vi "Gserver_main.vi"(8 "Database location":path=path "D:/Sgraph_database", 10 "debug":bool, 11 "DAQ-Queue":refnum<queue>) -> ()   [LabVIEW 2020, in "Sgraph_lib_V1.lvlib" / "Gserver.lvclass"]
doc: "Gserver service.\n\nThis service will act on Gviewer queries.\nThis VI must be started to enable the Sgraph functionality\n\nUse the Close method of the Gserver class after the main application is ended to free all resources."
uses:
  Gserver.lvclass
  controls/Typedef_Gserver-init.ctl
  HISW/controls/typedef-DAQ-datagram.ctl
  HISW/controls/typedef-Qtype.ctl
  C:/Sgraph/Sgraph/source/Vsolver/Vsolver.lvclass
  Gserver.lvclass/Gserver.ctl
  Common/controls/MeMapInfo.ctl
  Common/controls/MMap_element.ctl
  FAMM/controls/typedef-functions.ctl
  Gview/controls/Typedef_Live.ctl
  controls/Typedef_Sgraph_Query.ctl
  Gview/controls/Typedef_Gserver-Replies.ctl
  Gview/controls/Typedef_ServerActions.ctl
  FAMM/FAMM.lvclass/FAMM.ctl
  Gview/controls/Typedef_datarequest.ctl
  FAMM/FAMM.lvclass
  HISW/HISW.lvclass
  FAMM/controls/typedef_FAMM_Query.ctl
  Common/controls/Global-services.vi
  Vsolver/Vsolver.lvclass
  Builds/Sgraph_lib_V1.lvlib
  Gview/Gviewer.lvclass
panel:
  out "error out":errorcluster
  out "HISW-# elements in queue":i32
  out "HISW-iteration":i32
  out "# elements in queue":i32
  out "Graphs Running":string[](array[string])
  out "Gserver":picture
  out "GserverInitState":T1
  # "debug info"
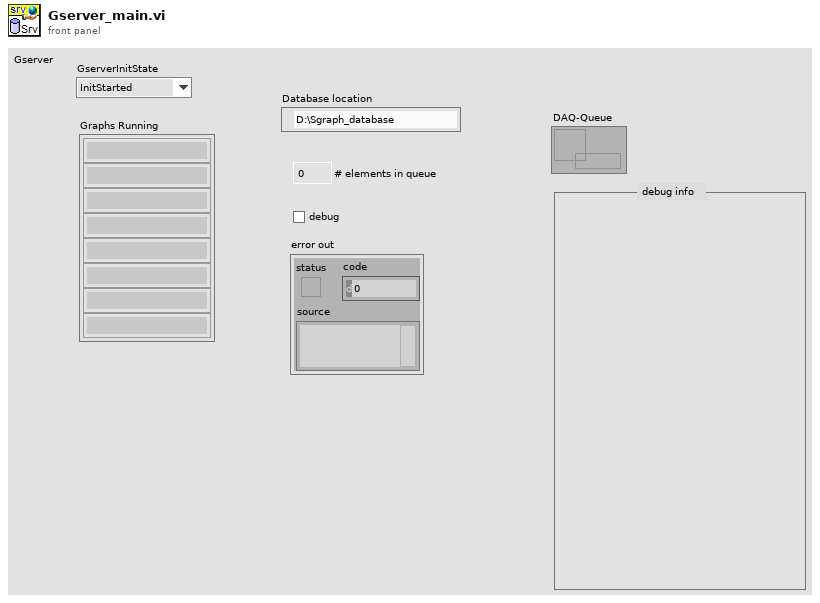
[diagram p1: front panel]
types:
  T1 = typedef "Sgraph_lib_V1.lvlib/Gserver.lvclass/Typedef_Gserver-init.ctl" = enum16{"InitStarted", "FAMM_started", "HISW_Started", "Active"}
  T2 = typedef "Sgraph_lib_V1.lvlib/typedef-functions.ctl" = enum16{"PAQ-request", "PAQ-taglist-request", "WAQ-request", "EAQ-request", "TAG-based-request", "PAQ-MemoryMap", "Exit-FAMM"}
  T3 = typedef "Sgraph_lib_V1.lvlib/MeMapInfo.ctl" = cluster{"MemLayer":T4[]}
  T4 = typedef "Sgraph_lib_V1.lvlib/MMap_element.ctl" = cluster{"Name":string, "Length":i32, "Pointer":i32, "Tbegin":dbl, "Tend":dbl, "Tmin":dbl, "Tmax":dbl, "Tpnt-1":dbl, "Tpnt":dbl, "Tpnt+1":dbl, "Array":dbl[]}
  T5 = typedef "Sgraph_lib_V1.lvlib/Gserver.lvclass/Typedef_Sgraph_Query.ctl" = cluster{"ViewportName":string, "Tags":string[], "Time-Start":timestamp, "Time-End":timestamp, "Pixels":i32, "Live":T6, "TimeSpan(sec)":dbl, "GViewer-Queue":refnum<queue>}
  T6 = typedef "Sgraph_lib_V1.lvlib/Gviewer.lvclass/Typedef_Live.ctl" = enum16{"Live View", "Freeze"}
  T7 = typedef "Sgraph_lib_V1.lvlib/Typedef_ServerActions.ctl" = enum16{"GraphUpdate", "SendAllTags", "SendIniPath", "SetGeneralOptions", "EditTagsOpen", "EditTagsPresetSave", "EditTagsPresetLoad", "EditTagsClose", "NewTagSelection", "ExitGraph"}
  T8 = typedef "Typedef_Gserver-Replies.ctl" = cluster{"ServerActions":T7, "data":variant, "Source":string, "Time Stamp":timestamp}
  T9 = typedef "Sgraph_lib_V1.lvlib/Gviewer.lvclass/Typedef_datarequest.ctl" = cluster{"Tags":string[], "Live":T6, "Time-Start":timestamp, "Time-End":timestamp, "TimeSpan":dbl, "DisplayResolution":i32}
  T10 = typedef "Sgraph_lib_V1.lvlib/typedef-Qtype.ctl" = enum16{"PAQ", "WAQ", "EAQ", "End-Service"}
  T11 = typedef "Sgraph_lib_V1.lvlib/typedef-DAQ-datagram.ctl" = cluster{"Time Stamp":timestamp, "Source":string, "Data":variant, "Qtype":T10}
  T12 = typedef "typedef_FAMM_Query.ctl" = cluster{"Time Stamp":timestamp, "FAMM-function":T2, "Source":string, "Data":variant}
  T13 = typedef "Sgraph_lib_V1.lvlib/Gserver.lvclass/Typedef_Gviewer-Query.ctl" = cluster{"Query_type":T14, "data":variant, "Source":string, "Time Stamp":timestamp}
  T14 = typedef "Sgraph_lib_V1.lvlib/Gserver.lvclass/Typedef_QueryType.ctl" = enum16{"Subscribe", "DataRequest", "RequestAllTags", "RequestIniPath", "FAMMstarted", "SetClientOptions", "GviewerUpdate", "OpenNewGraph", "CloseClient", "CloseAllClients", "Close Gserver", "OpenMemoryMap", "MeMapDataRequest", "MeMapDataResponse"}
  T15 = typedef "Sgraph_lib_V1.lvlib/FAMM.lvclass/Typedef_Gviewer_TagsUnits.ctl" = cluster{"PAQ_TAGs":string[], "WAQ_TAGs":string[], "EAQ_TAGs":string[], "PAQtagProps":T16[], "WAQtagProps":T16[], "EAQtagProps":T16[]}
  T16 = typedef "Sgraph_lib_V1.lvlib/typedef_com_TagProp.ctl" = cluster{"Description":string, "EngUnits":string, "RangeH":dbl, "RangeL":dbl, "Resolution":i32, "Obsolete":bool, "ChangeDate":timestamp, "ChangeSource":string, "ChangeReason":string, "TagFunc":u32}
  T17 = cluster{"FAMM_PAQ_Layers":i32, "FAMM_PAQ_resolution":dbl}
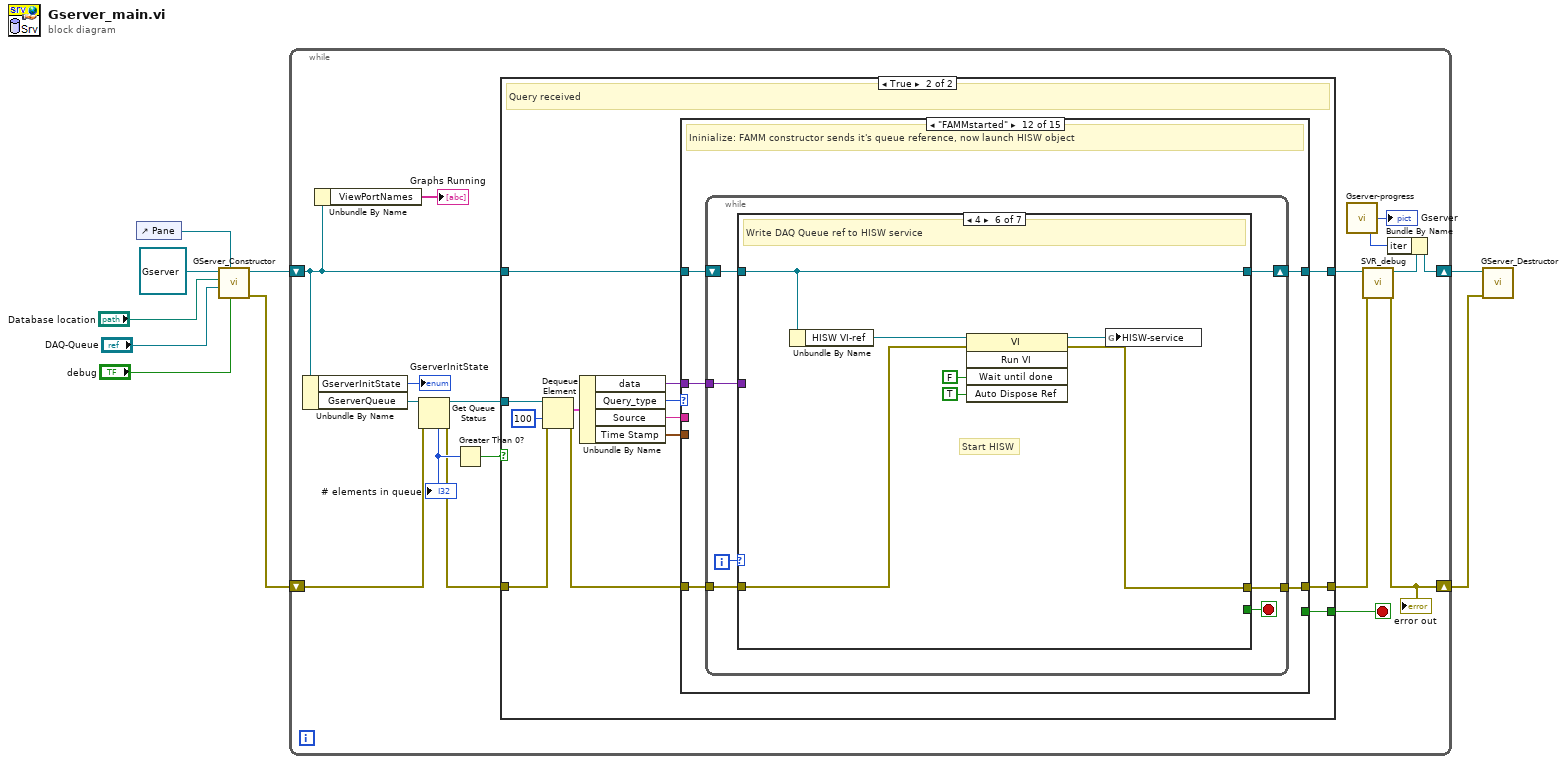
[diagram p0: block diagram]
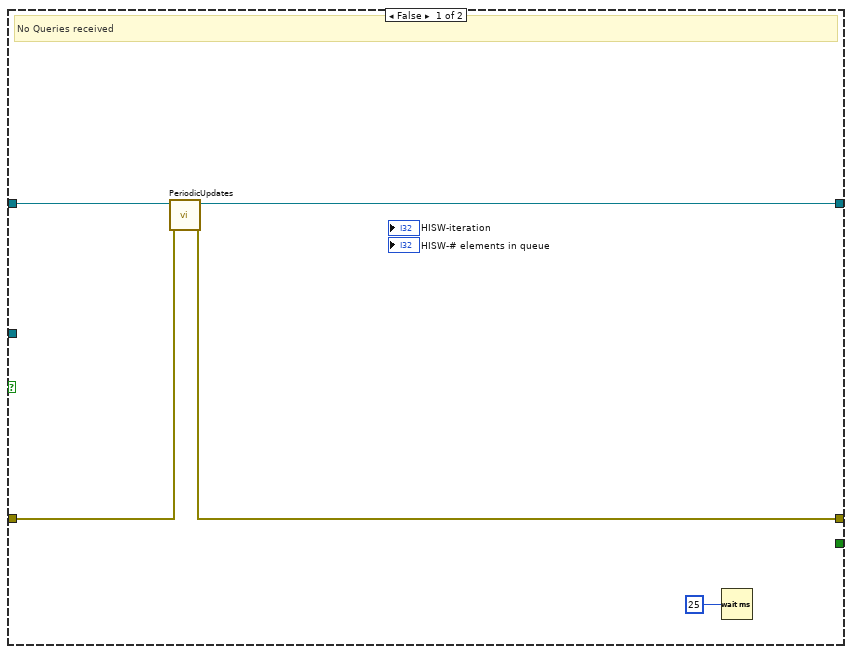
[diagram p2: hidden frame]
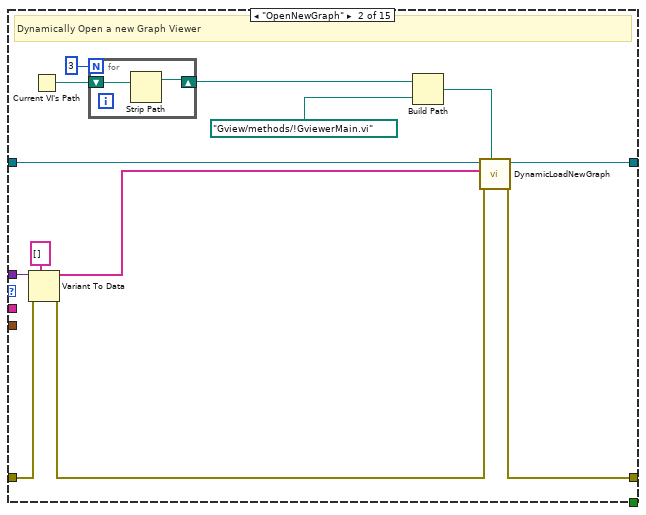
[diagram p4: hidden frame]
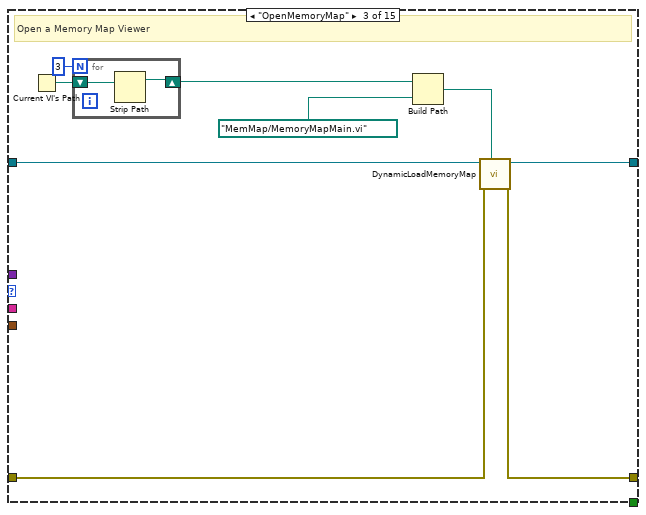
[diagram p5: hidden frame]
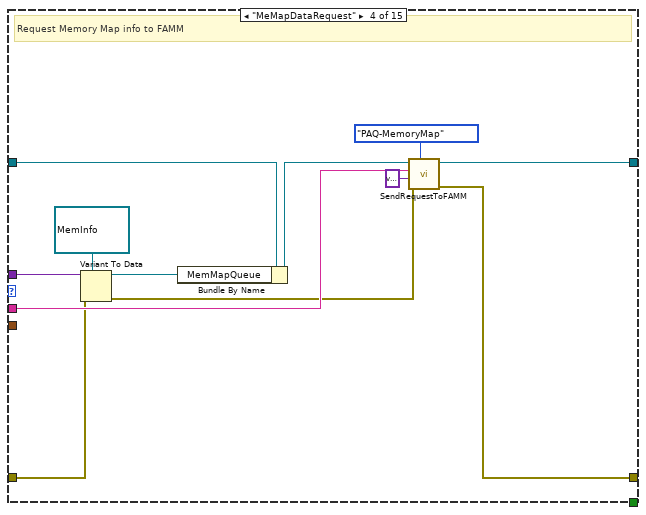
[diagram p6: hidden frame]
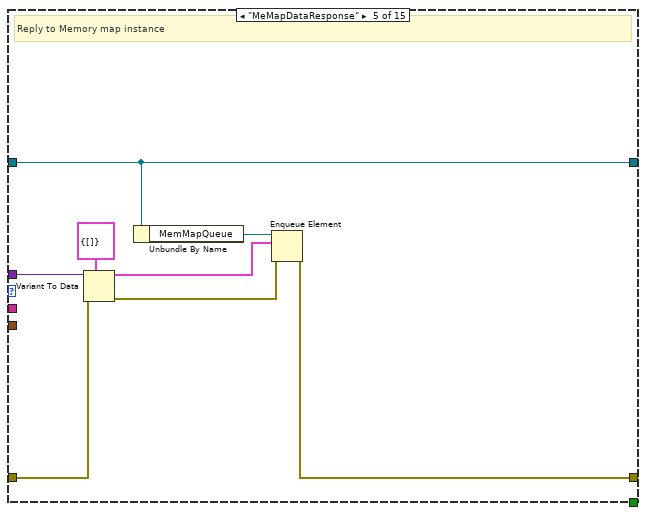
[diagram p7: hidden frame]
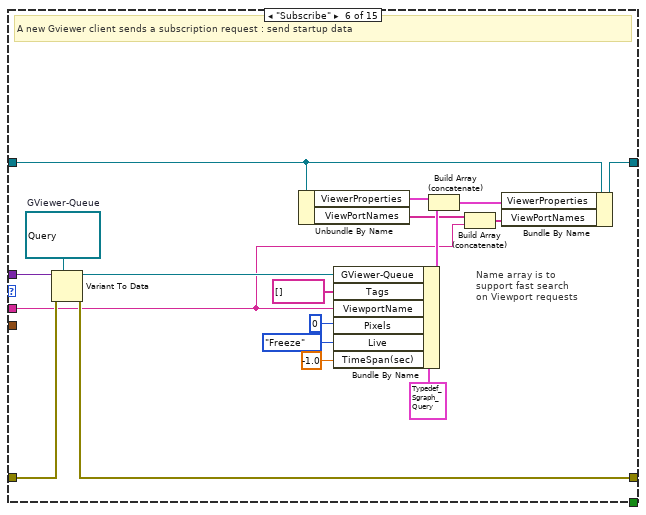
[diagram p8: hidden frame]
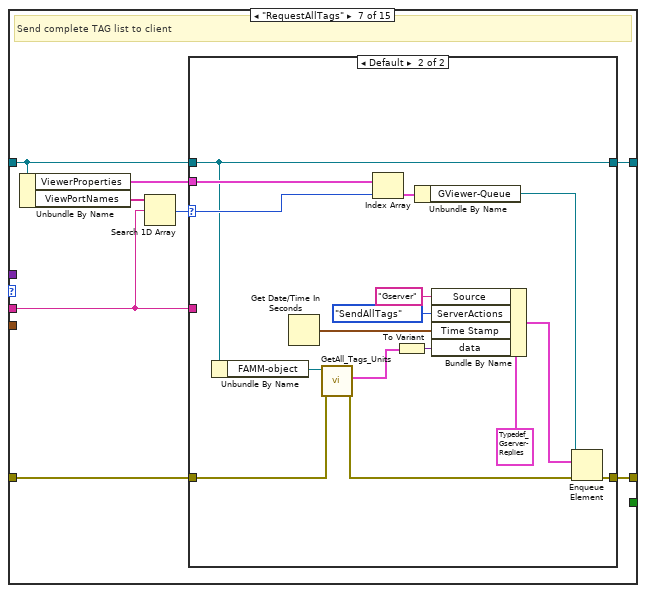
[diagram p9: hidden frame]
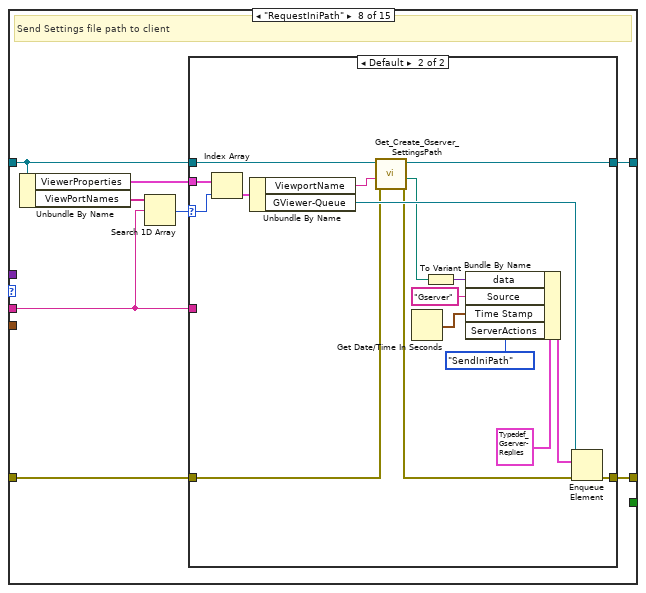
[diagram p11: hidden frame]
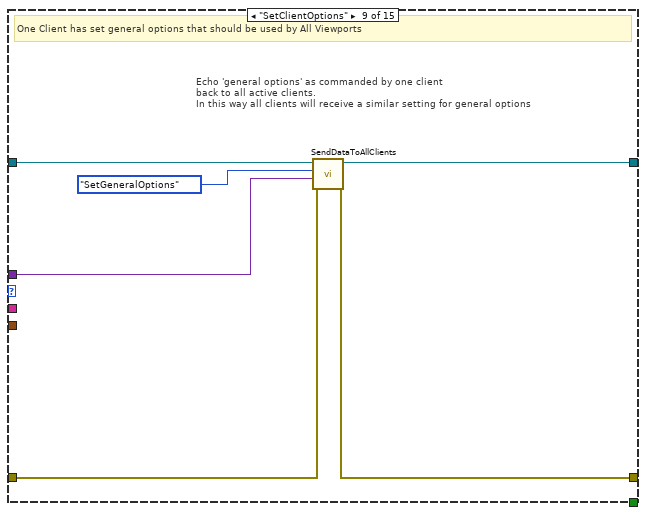
[diagram p13: hidden frame]
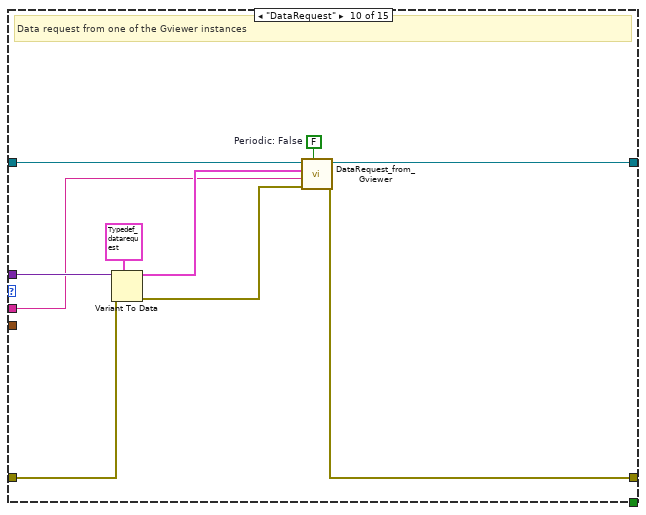
[diagram p14: hidden frame]
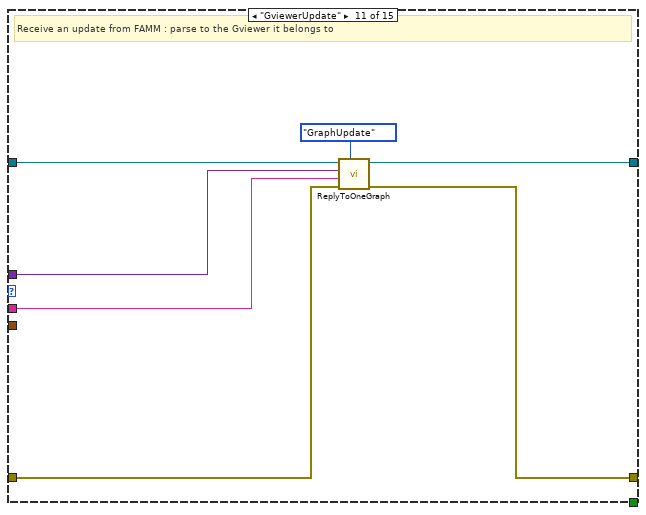
[diagram p15: hidden frame]
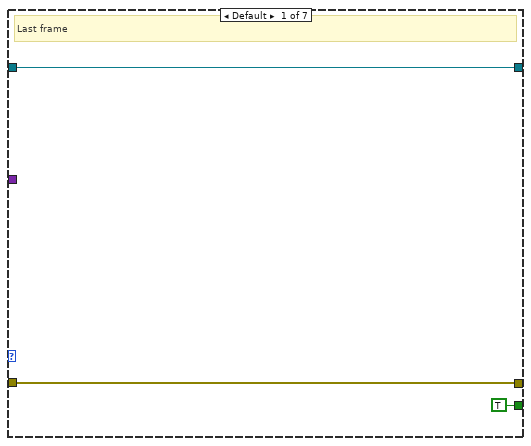
[diagram p16: hidden frame]
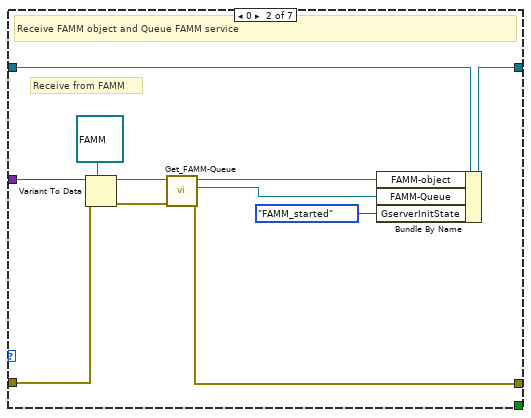
[diagram p17: hidden frame]
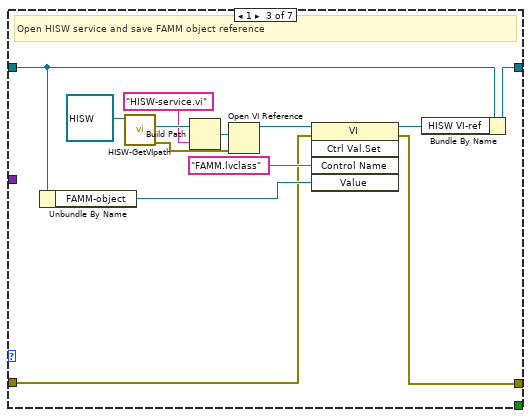
[diagram p18: hidden frame]
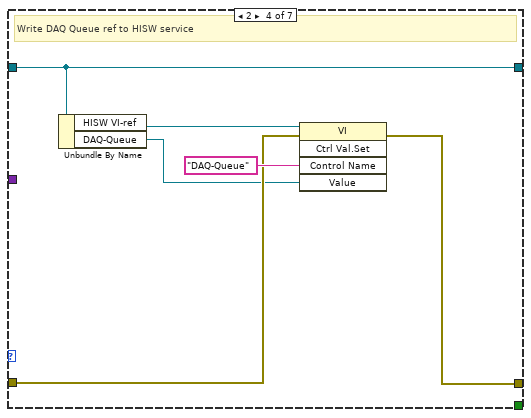
[diagram p19: hidden frame]
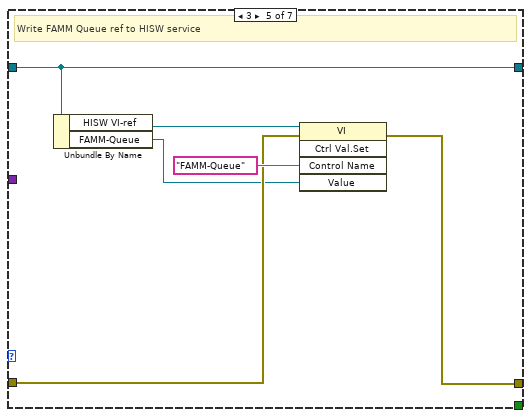
[diagram p20: hidden frame]
diagram:
  n1 = control-ref of="Pane"() -> (w1:refnum<vi>)
  n2 = call "GServer_Constructor.vi"("Debug"="debug", "Pane"=w1, "DAQ-Queue"="DAQ-Queue", "Database location"="Database location", "Gserver in"=refnum<class "Gserver.lvclass"> refnum) -> ("error out"=w8:errorcluster, "Gserver out"=w9:refnum<class "Gserver.lvclass">)  [unwired: 5 in]
  n3 = while {
    shift-right: [w15] -> w7
    shift-left: w9 -> [w17]
    shift-right: [w10] -> w6
    shift-left: w8 -> [w22]
    stop <- w18 stop-if-true
    n4 = Unbundle By Name(w17) -> ("GserverInitState"=→"GserverInitState":T1, "GserverQueue"=w26:refnum<queue>)
    n5 = Unbundle By Name(w17) -> ("ViewPortNames"=→"Graphs Running":string[])
    n6 = Get Queue Status(queue=w26, error in (no error)=w22) -> (queue out=w23:refnum<queue>, error out=w21:errorcluster, # elements in queue=w25:i32)  [unwired: 1 in, 5 out]
    "# elements in queue" <- w25
    n7 = Greater Than 0?(x=w25) -> (x > 0?=w24:bool)
    n8 = case shown="True" w24 {
      tunnel: w17 -> [w30 w38]
      tunnel: w21 -> [w29 w42]
      tunnel: [w28 w36] -> w13
      tunnel: [w27 w37] -> w11
      tunnel: w23 -> [_ w44]
      tunnel: [_ w33] -> w18
      frame False {
        # "No Queries received"
        n9 = call "PeriodicUpdates.vi"("error in (no error)"=w29, "Gserver in"=w30) -> ("error out"=w27:errorcluster, "Gserver out"=w28:refnum<class "Gserver.lvclass">)  [unwired: 8 in]
        n10 = Wait (ms)(milliseconds to wait=u32 25) -> ()  [unwired: 1 out]
      }
      frame True {
        # "Query received"
        n11 = Dequeue Element(queue=w44, timeout in ms (-1)=100, error in (no error)=w42) -> (element=w41:T13, error out=w39:errorcluster)  [unwired: 2 out]
        n12 = Unbundle By Name(w41) -> ("data"=w35:variant, "Query_type"=w40:T14, "Source"=w32:string, "Time Stamp"=w34:timestamp)
        n13 = case shown="\"FAMMstarted\"" w40 {
          tunnel: w39 -> [w45 w47 w63 w74 w85 w96 w114 w140 w165 w177 w182 w188 w255 w261 w272]
          tunnel: w38 -> [w46 w52 w65 w81 w92 w110 w116 w142 w169 w175 w186 w190 w257 w260 w271]
          tunnel: [w45 w51 w64 w75 w86 w97 w113 w139 w164 w171 w184 w187 w254 w258 w269] -> w37
          tunnel: [w46 w53 w66 w78 w92 w109 w115 w141 w168 w176 w185 w191 w256 w259 w270] -> w36
          tunnel: w35 -> [_ w59 _ w84 w90 w100 _ _ w166 w179 w180 w189 _ _ _]
          tunnel: w34 -> [_ _ _ _ _ _ _ _ _ _ _ _ _ _ _]
          tunnel: [_ _ _ _ _ _ _ _ _ _ _ _ _ _ w268] -> w33
          tunnel: w32 -> [_ _ _ w77 _ w93 w117 w143 _ w172 w183 _ w253 _ _]
          frame Default {
            # "Not implemented"
          }
          frame "OpenNewGraph" {
            # "Dynamically Open a new Graph Viewer"
            n14 = Variant To Data(error in=w47, type=string[] [], Variant=w59) -> (data=w49:string[], error out=w48:errorcluster)
            n15 = Current VI's Path() -> (path=w57:path)
            n16 = for {
              N: 3 -> [_]
              shift-right: [w60] -> w55
              shift-left: w57 -> [w61]
              n17 = Strip Path(path=w61) -> (stripped path=w60:path)  [unwired: 1 out]
            }
            n18 = Build Path(base path=w55, name or relative path=path "Gview/methods/!GviewerMain.vi") -> (appended path=w50:path)
            n19 = call "DynamicLoadNewGraph.vi"("ViewerPath"=w50, "error in (no error)"=w48, "Preferred_tags"=w49, "Gserver in"=w52) -> ("error out"=w51:errorcluster, "Gserver out"=w53:refnum<class "Gserver.lvclass">)  [unwired: 6 in]
          }
          frame "OpenMemoryMap" {
            # "Open a Memory Map Viewer"
            n20 = Current VI's Path() -> (path=w70:path)
            n21 = for {
              N: 3 -> [_]
              shift-right: [w71] -> w68
              shift-left: w70 -> [w72]
              n22 = Strip Path(path=w72) -> (stripped path=w71:path)  [unwired: 1 out]
            }
            n23 = Build Path(base path=w68, name or relative path=path "MemMap/MemoryMapMain.vi") -> (appended path=w62:path)
            n24 = call "DynamicLoadMemoryMap.vi"("ApplicationPath"=w62, "error in (no error)"=w63, "Gserver in"=w65) -> ("error out"=w64:errorcluster, "Gserver out"=w66:refnum<class "Gserver.lvclass">)  [unwired: 7 in]
          }
          frame "MeMapDataRequest" {
            # "Request Memory Map info to FAMM"
            n25 = Variant To Data(error in=w74, type=refnum<queue> refnum ("queue out"), Variant=w84) -> (data=w82:refnum<queue>, error out=w76:errorcluster)
            n26 = Bundle By Name(cluster=w81, "MemMapQueue"=w82) -> (w79:refnum<class "Gserver.lvclass">)
            n27 = call "SendRequestToFAMM.vi"("FAMM-function"=typedef-functions."PAQ-MemoryMap", "error in (no error)"=w76, "Data"=variant, "Source"=w77, "Gserver in"=w79) -> ("error out"=w75:errorcluster, "Gserver out"=w78:refnum<class "Gserver.lvclass">)  [unwired: 5 in]
          }
          frame "MeMapDataResponse" {
            # "Reply to Memory map instance"
            n28 = Variant To Data(error in=w85, type=T3 {"MemLayer"=[]} ("element"), Variant=w90) -> (data=w87:T3, error out=w88:errorcluster)
            n29 = Unbundle By Name(w92) -> ("MemMapQueue"=w91:refnum<queue>)
            n30 = Enqueue Element(queue=w91, element=w87, error in (no error)=w88) -> (error out=w86:errorcluster)  [unwired: 1 in, 2 out]
          }
          frame "Subscribe" {
            w101 = refnum<queue> refnum  # GViewer-Queue
            # "Name array is to\nsupport fast search\non Viewport requests"
            # "A new Gviewer client sends a subscription request : send startup data"
            n31 = Variant To Data(error in=w96, type=w101, Variant=w100) -> (data=w99:refnum<queue>, error out=w97:errorcluster)
            n32 = Unbundle By Name(w110) -> ("ViewerProperties"=w108:T5[], "ViewPortNames"=w95:string[])
            n33 = Bundle By Name(cluster=T5 {"ViewportName"="", "Tags"=[], "Time-Start"=timestamp(0 s since 1904-01-01), "Time-End"=timestamp(0 s since 1904-01-01), "Pixels"=0, "Live"=enum."Live View", "TimeSpan(sec)"=0.0, "GViewer-Queue"=refnum} ("Query_datagram"), "GViewer-Queue"=w99, "Tags"=string[] [], "ViewportName"=w93, "Pixels"=0, "Live"=Typedef_Live."Freeze", "TimeSpan(sec)"=-1.0) -> (w105:T5)
            n34 = Build Array (concatenate)(w108, w105) -> (w107:T5[])
            n35 = Build Array (concatenate)(w95, w93) -> (w94:string[])
            n36 = Bundle By Name(cluster=w110, "ViewerProperties"=w107, "ViewPortNames"=w94) -> (w109:refnum<class "Gserver.lvclass">)
          }
          frame "RequestAllTags" {
            # "Send complete TAG list to client"
            n37 = Unbundle By Name(w116) -> ("ViewerProperties"=w112:T5[], "ViewPortNames"=w118:string[])
            n38 = Search 1D Array(1D array=w118, element=w117) -> (index of element=w111:i32)  [unwired: 1 in]
            n39 = case shown="Default" w111 {
              selector: w111 -> [_ w135]
              tunnel: w117 -> [_ _]
              tunnel: w116 -> [w120 w131]
              tunnel: [w120 w131] -> w115
              tunnel: w114 -> [w119 w123]
              tunnel: [w119 w132] -> w113
              tunnel: w112 -> [_ w136]
              frame -1 {
              }
              frame Default {
                n40 = Unbundle By Name(w131) -> ("FAMM-object"=w124:refnum<class "FAMM.lvclass">)
                n41 = Get Date/Time In Seconds() -> (seconds since 1Jan1904=w127:timestamp)
                n42 = call "GetAll_Tags_Units.vi"("error in (no error)"=w123, "FAMM in"=w124) -> ("error out"=w122:errorcluster, "Tags_Units"=w121:T15)  [unwired: 7 in, 1 out]
                n43 = Index Array(array=w136, index=w135) -> (element=w134:T5)
                n44 = To Variant(anything=w121) -> (Variant=w125:variant)
                n45 = Unbundle By Name(w134) -> ("GViewer-Queue"=w133:refnum<queue>)
                n46 = Bundle By Name(cluster=T8 {"ServerActions"=enum."GraphUpdate", "data"=variant, "Source"="", "Time Stamp"=timestamp(0 s since 1904-01-01)} ("element"), "Source"="Gserver", "ServerActions"=Typedef_ServerActions."SendAllTags", "Time Stamp"=w127, "data"=w125) -> (w129:T8)
                n47 = Enqueue Element(queue=w133, element=w129, error in (no error)=w122) -> (error out=w132:errorcluster)  [unwired: 1 in, 2 out]
              }
            }
          }
          frame "RequestIniPath" {
            # "Send Settings file path to client"
            n48 = Unbundle By Name(w142) -> ("ViewerProperties"=w138:T5[], "ViewPortNames"=w144:string[])
            n49 = Search 1D Array(1D array=w144, element=w143) -> (index of element=w137:i32)  [unwired: 1 in]
            n50 = case shown="Default" w137 {
              selector: w137 -> [_ w162]
              tunnel: w143 -> [_ _]
              tunnel: w142 -> [w146 w154]
              tunnel: [w146 w155] -> w141
              tunnel: w140 -> [w145 w151]
              tunnel: [w145 w159] -> w139
              tunnel: w138 -> [_ w163]
              frame -1 {
              }
              frame Default {
                n51 = Index Array(array=w163, index=w162) -> (element=w161:T5)
                n52 = Unbundle By Name(w161) -> ("ViewportName"=w153:string, "GViewer-Queue"=w160:refnum<queue>)
                n53 = call "Get_Create_Gserver_SettingsPath.vi"("error in (no error)"=w151, "ViewPortName"=w153, "Gserver in"=w154) -> ("error out"=w152:errorcluster, "Viewport settings path"=w147:path, "Gserver out"=w155:refnum<class "Gserver.lvclass">)  [unwired: 6 in]
                n54 = Get Date/Time In Seconds() -> (seconds since 1Jan1904=w149:timestamp)
                n55 = To Variant(anything=w147) -> (Variant=w150:variant)
                n56 = Bundle By Name(cluster=T8 {"ServerActions"=enum."GraphUpdate", "data"=variant, "Source"="", "Time Stamp"=timestamp(0 s since 1904-01-01)} ("element"), "data"=w150, "Source"="Gserver", "Time Stamp"=w149, "ServerActions"=Typedef_ServerActions."SendIniPath") -> (w157:T8)
                n57 = Enqueue Element(queue=w160, element=w157, error in (no error)=w152) -> (error out=w159:errorcluster)  [unwired: 1 in, 2 out]
              }
            }
          }
          frame "SetClientOptions" {
            # "Echo 'general options' as commanded by one client\nback to all active clients.\nIn this way all clients will receive a similar setting for general options"
            # "One Client has set general options that should be used by All Viewports"
            n58 = call "SendDataToAllClients.vi"("error in (no error)"=w165, "data"=w166, "ServerActions"=Typedef_ServerActions."SetGeneralOptions", "Gserver in"=w169) -> ("error out"=w164:errorcluster, "Gserver out"=w168:refnum<class "Gserver.lvclass">)  [unwired: 6 in]
          }
          frame "DataRequest" {
            w170 = FALSE  # Periodic: False
            # "Data request from one of the Gviewer instances"
            n59 = Variant To Data(error in=w177, type=T9 {"Tags"=[], "Live"=enum."Live View", "Time-Start"=timestamp(0 s since 1904-01-01), "Time-End"=timestamp(0 s since 1904-01-01), "TimeSpan"=0.0, "DisplayResolution"=0} ("Cluster"), Variant=w179) -> (data=w174:T9, error out=w173:errorcluster)
            n60 = call "DataRequest_from_Gviewer.vi"("Periodic?"=w170, "error in (no error)"=w173, "Sending Gviewer"=w172, "DataRequest"=w174, "Gserver in"=w175) -> ("error out"=w171:errorcluster, "Gserver out"=w176:refnum<class "Gserver.lvclass">)  [unwired: 5 in]
          }
          frame "GviewerUpdate" {
            # "Receive an update from FAMM : parse to the Gviewer it belongs to"
            n61 = call "ReplyToOneGraph.vi"("ServerActions"=Typedef_ServerActions."GraphUpdate", "error in (no error)"=w182, "Graph name"=w183, "data"=w180, "Gserver in"=w186) -> ("error out"=w184:errorcluster, "Gserver out"=w185:refnum<class "Gserver.lvclass">)  [unwired: 5 in]
          }
          frame "FAMMstarted" {
            # "Ininialize: FAMM constructor sends it's queue reference, now launch HISW object"
            n62 = while {
              tunnel: w189 -> [w196]
              tunnel: w188 -> [w195]
              shift-right: [w198] -> w191
              shift-left: w190 -> [w197]
              tunnel: [w192] -> w187
              i -> [w194]
              stop <- w193 stop-if-true
              n63 = case shown="4" w194 {
                tunnel: [w201 w212 w215 w229 w235 w244 w246] -> w198
                tunnel: w197 -> [w201 w210 w214 w229 w235 w244 w245]
                tunnel: w196 -> [_ w209 _ _ _ _ _]
                tunnel: w195 -> [w199 w208 w217 w230 w236 w240 w250]
                tunnel: [TRUE _ _ _ _ _ _] -> w193
                tunnel: [w199 w204 w213 w226 w232 w239 w251] -> w192
                frame Default {
                  # "Last frame"
                }
                frame 0 {
                  # "Receive from FAMM"
                  # "Receive FAMM object and Queue FAMM service"
                  n64 = Variant To Data(error in=w208, type=refnum<class "FAMM.lvclass"> refnum ("FAMM out"), Variant=w209) -> (data=w206:refnum<class "FAMM.lvclass">, error out=w205:errorcluster)
                  n65 = call-dynamic "Get_FAMM-Queue.vi"("error in (no error)"=w205, "FAMM in"=w206) -> ("error out"=w204:errorcluster, "FAMM-Queue"=w202:refnum<queue>, "FAMM out"=w203:refnum<class "FAMM.lvclass">)  [unwired: 7 in]
                  n66 = Bundle By Name(cluster=w210, "FAMM-object"=w203, "FAMM-Queue"=w202, "GserverInitState"=Typedef_Gserver-init."FAMM_started") -> (w212:refnum<class "Gserver.lvclass">)
                }
                frame 1 {
                  # "Open HISW service and save FAMM object reference"
                  n67 = Unbundle By Name(w214) -> ("FAMM-object"=w218:refnum<class "FAMM.lvclass">)
                  n68 = call "HISW-GetVIpath.vi"("HISW in"=refnum<class "HISW.lvclass"> refnum) -> ("error out"=w223:errorcluster, "MethodsPath"=w224:path)  [unwired: 8 in, 1 out]
                  n69 = Build Path(base path=w224, name or relative path="HISW-service.vi") -> (appended path=w225:path)
                  n70 = Open VI Reference(vi path=w225, error in (no error)=w223) -> (vi reference=w222:refnum<vi>)  [unwired: 4 in, 1 out]
                  n71 = invoke class="VI" method="Ctrl Val.Set"(reference=w222, error in=w217, "Control Name"="FAMM.lvclass", "Value"=w218) -> (reference out=w216:refnum<vi>, error out=w213:errorcluster)  [unwired: 1 in, 3 out]
                  n72 = Bundle By Name(cluster=w214, "HISW VI-ref"=w216) -> (w215:refnum<class "Gserver.lvclass">)
                }
                frame 2 {
                  # "Write DAQ Queue ref to HISW service"
                  n73 = Unbundle By Name(w229) -> ("HISW VI-ref"=w228:refnum<vi>, "DAQ-Queue"=w227:refnum<queue>)
                  n74 = invoke class="VI" method="Ctrl Val.Set"(reference=w228, error in=w230, "Control Name"="DAQ-Queue", "Value"=w227) -> (error out=w226:errorcluster)  [unwired: 1 in, 4 out]
                }
                frame 3 {
                  # "Write FAMM Queue ref to HISW service"
                  n75 = Unbundle By Name(w235) -> ("HISW VI-ref"=w234:refnum<vi>, "FAMM-Queue"=w233:refnum<queue>)
                  n76 = invoke class="VI" method="Ctrl Val.Set"(reference=w234, error in=w236, "Control Name"="FAMM-Queue", "Value"=w233) -> (error out=w232:errorcluster)  [unwired: 1 in, 4 out]
                }
                frame 4 {
                  # "Start HISW"
                  # "Write DAQ Queue ref to HISW service"
                  n77 = Unbundle By Name(w244) -> ("HISW VI-ref"=w241:refnum<vi>)
                  n78 = invoke class="VI" method="Run VI"(reference=w241, error in=w240, "Wait until done"=FALSE ("Wait Until Done"), "Auto Dispose Ref"=TRUE ("Auto Dispose Reference")) -> (reference out=w238:refnum<vi>, error out=w239:errorcluster)  [unwired: 1 in, 3 out]
                  n79 = global write "Global-services.vi" "HISW-service"(w238) -> ()
                }
                frame 5 {
                  # "Get FAMM PAQ resolution data"
                  n80 = Unbundle By Name(w245) -> ("FAMM-object"=w252:refnum<class "FAMM.lvclass">)
                  n81 = call "GetPAQresolution.vi"("error in (no error)"=w250, "FAMM in"=w252) -> ("error out"=w251:errorcluster, "PAQ-resolution"=w249:T17)  [unwired: 7 in, 1 out]
                  n82 = Unbundle By Name(w249) -> ("FAMM_PAQ_Layers"=w248:i32, "FAMM_PAQ_resolution"=w247:dbl)
                  n83 = Bundle By Name(cluster=w245, "FAMM_PAQ_Layers"=w248, "FAMM_PAQ_resolution"=w247) -> (w246:refnum<class "Gserver.lvclass">)
                }
              }
            }
          }
          frame "CloseClient" {
            # "Graph display request to close the graph"
            n84 = call "CloseOneGraph.vi"("error in (no error)"=w255, "Graph name"=w253, "Gserver in"=w257) -> ("error out"=w254:errorcluster, "Gserver out"=w256:refnum<class "Gserver.lvclass">)  [unwired: 7 in]
          }
          frame "CloseAllClients" {
            # "One Graph display requests to close all Graphs"
            n85 = Unbundle By Name(w260) -> ("ViewPortNames"=w262:string[])
            n86 = for "Loop over all viewports and perform a clean Graph Close" {
              tunnel: w262 -> [w266] mode=indexing
              shift-right: [w263] -> w259
              shift-left: w260 -> [w267]
              shift-right: [w264] -> w258
              shift-left: w261 -> [w265]
              n87 = call "CloseOneGraph.vi"("error in (no error)"=w265, "Graph name"=w266, "Gserver in"=w267) -> ("error out"=w264:errorcluster, "Gserver out"=w263:refnum<class "Gserver.lvclass">)  [unwired: 7 in]
            }
          }
          frame "Close Gserver" {
            # "Close the SGraph server"
            n88 = while {
              shift-right: [w276] -> w269
              shift-left: w272 -> [w277]
              shift-right: [w274] -> w270
              shift-left: w271 -> [w275]
              tunnel: [w273] -> w268
              i -> [w278]
              stop <- w273 stop-if-true
              n89 = case shown="1" w278 {
                tunnel: [TRUE _ _ _] -> w273
                tunnel: w277 -> [w280 w291 w299 w302]
                tunnel: [w280 w289 w298 w303] -> w276
                tunnel: w275 -> [w279 w292 w301 w305]
                tunnel: [w279 w283 w301 w306] -> w274
                frame Default {
                  # "Last frame: no code here"
                }
                frame 0 {
                  # "Close Vsolver class, End HISW service"
                  n90 = call "Vsolver_destructor.vi"("error in (no error)"=w291, "Vsolver in"=w292) -> ("error out"=w290:errorcluster, "Vsolver out"=w283:refnum<class "Gserver.lvclass">)  [unwired: 8 in]
                  n91 = Get Date/Time In Seconds() -> (seconds since 1Jan1904=w287:timestamp)
                  n92 = Unbundle By Name(w283) -> ("DAQ-Queue"=w282:refnum<queue>)
                  n93 = Bundle By Name(cluster=T11 {"Time Stamp"=timestamp(0 s since 1904-01-01), "Source"="", "Data"=variant, "Qtype"=enum."PAQ"} ("element"), "Time Stamp"=w287, "Source"="Gserver", "Qtype"=typedef-Qtype."End-Service") -> (w284:T11)
                  n94 = Enqueue Element(queue=w282, element=w284, error in (no error)=w290) -> (error out=w289:errorcluster)  [unwired: 1 in, 2 out]
                }
                frame 1 {
                  # "Exit FAMM service"
                  n95 = Get Date/Time In Seconds() -> (seconds since 1Jan1904=w296:timestamp)
                  n96 = Bundle By Name(cluster=T12 {"Time Stamp"=timestamp(0 s since 1904-01-01), "FAMM-function"=enum."PAQ-request", "Source"="", "Data"=variant} ("element"), "FAMM-function"=typedef-functions."Exit-FAMM", "Source"="Gserver", "Time Stamp"=w296) -> (w293:T12)
                  n97 = Unbundle By Name(w301) -> ("FAMM-Queue"=w300:refnum<queue>)
                  n98 = Enqueue Element(queue=w300, element=w293, error in (no error)=w299) -> (error out=w298:errorcluster)  [unwired: 1 in, 2 out]
                }
                frame 2 {
                  # "Exit Viewport Applications"
                  n99 = call "SendDataToAllClients.vi"("error in (no error)"=w302, "ServerActions"=Typedef_ServerActions."ExitGraph", "Gserver in"=w305) -> ("error out"=w303:errorcluster, "Gserver out"=w306:refnum<class "Gserver.lvclass">)  [unwired: 7 in]
                }
              }
            }
          }
        }
      }
    }
    n100 = call "Gserver-progress.vi"() -> ("37x37"=→"Gserver":picture, "iter"=w14:u64)  [unwired: 6 in]
    n101 = call "SVR_debug.vi"("error in (no error)"=w11, "Gserver in"=w13) -> ("error out"=w10:errorcluster, "Gserver out"=w12:refnum<class "Gserver.lvclass">)  [unwired: 8 in]
    "error out" <- w10
    n102 = Bundle By Name(cluster=w12, "iter"=w14) -> (w15:refnum<class "Gserver.lvclass">)
  }
  n103 = call "GServer_Destructor.vi"("error in (no error)"=w6, "Gserver in"=w7) -> ()  [unwired: 8 in, 2 out]
